vi "zero.vi"(8 "error in (no error)":errorcluster, 11 "NI-9237 in":refnum<class "NI-9237.lvclass">) -> (0 "error out":errorcluster, 3 "NI-9237 out":refnum<class "NI-9237.lvclass">)   [LabVIEW 2025, in "Wheatstone Bridge.lvlib" / "NI-9237.lvclass"]
uses:
  NI-9237.lvclass
  NI-9237.lvclass/NI-9237.ctl
  <vilib>/DAQmx/read.llb/DAQmx Read (Analog DBL 1Chan 1Samp).vi
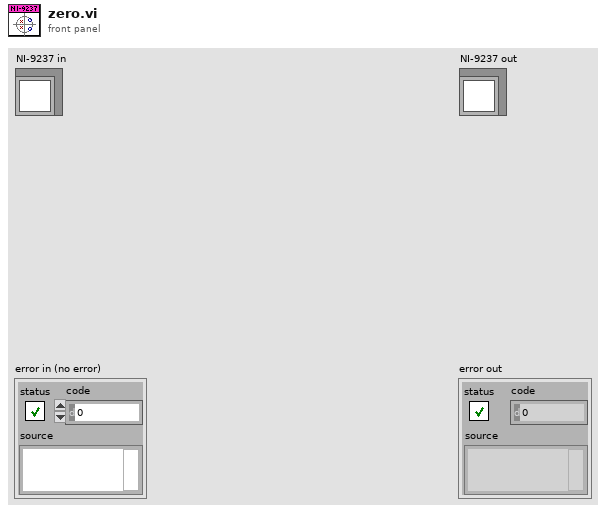
[diagram p1: front panel]
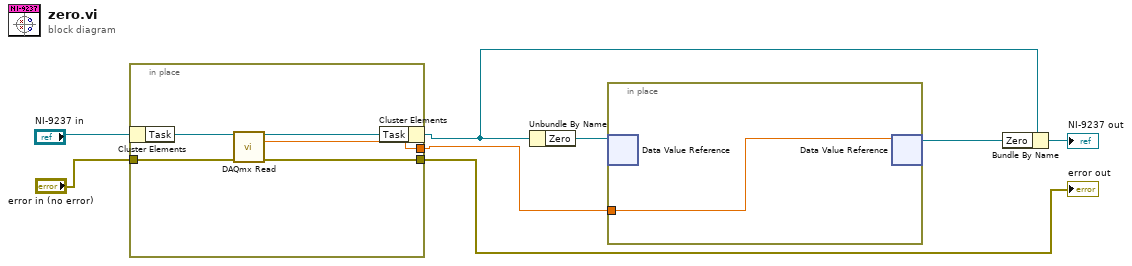
[diagram p0: block diagram]
diagram:
  n1 = in-place {
    in-place-border: [w11] -> w3
    in-place-border: "error in (no error)" -> [w10]
    in-place-border: [w9] -> w1
    n2 = in-place-cluster #1("NI-9237 in") -> ("Task"=w13:refnum<k21>)
    n3 = call-poly <vilib>:"DAQmx Read.vi"("task/channels in"=w13, "error in"=w10) -> ("task out"=w12:refnum<k21>, "data"=w9:dbl, "error out"=w11:errorcluster)  [unwired: 11 in]
    n4 = in-place-cluster #1("Task"=w12) -> (w4:refnum<class "NI-9237.lvclass">)
  }
  "error out" <- w3
  n5 = Unbundle By Name(w4) -> ("Zero"=w8:refnum<data-value>)
  n6 = in-place {
    in-place-border: w1 -> [w14]
    n7 = in-place-dvr #2(w8) -> ()  [unwired: 2 out]
    n8 = in-place-dvr #2(w14) -> (w6:refnum<data-value>)  [unwired: 1 out]
  }
  n9 = Bundle By Name(cluster=w4, "Zero"=w6) -> (→"NI-9237 out":refnum<class "NI-9237.lvclass">)
